vi "test tools list schema details.vi"(8 "error in (no error)":errorcluster) -> (0 "error out":errorcluster, 3 "body":string)   [LabVIEW 2020, in "MCP Server tests.lvlib"]
doc: "tools/list must describe every input completely enough for strict clients such as ChatGPT/Codex. fake_tool_schema_shapes and fake_tool_array_shapes are found by their MCP names, and each kind of input gets its own assertion: a timestamp is a string with format date-time, also as array element; a cluster is an object with properties named by the element labels, nested to any depth and inside arrays; an array of variants (no JSON type) has items {}; a 2D array is an array of arrays; an enum is a string whose enum lists the item names. The request is sent with the LabVIEW HTTP Client directly."
uses:
  MCP Server tests.lvlib
  facb51cd-7822-4ca8-a256-520732c48ef2.vi
  7ce273db-93f1-4574-9673-25cb3b7d48c6.vi
  <vilib>/JDP Science/JSONtext/Next JSON Value.vi
  <vilib>/JDP Science/JSONtext/String Subset.vi
  <vilib>/JDP Science/JSONtext/Parsing/Advance past next JSON Value (inlined COPY).vi
  <vilib>/JDP Science/JSONtext/Parsing/Advance past whitespace.vi
  <vilib>/JDP Science/JSONtext/Parsing/Advance past String.vi
  <vilib>/JDP Science/JSONtext/Parsing/Advance past Number.vi
  <vilib>/JDP Science/JSONtext/Parsing/Advance past Line Ending.vi
  <vilib>/JDP Science/JSONtext/Parsing/Parse Full Path or Item Name.vi
  <vilib>/JDP Science/JSONtext/Parsing/Advance past Array.vi
  <vilib>/JDP Science/JSONtext/Parsing/Advance past Object.vi
  <vilib>/JDP Science/JSONtext/support/Error Cluster From Code.vi
  <vilib>/JDP Science/JSONtext/Offset/Find Item Locations by Path.vi
  <vilib>/JDP Science/JSONtext/JSON text to Variant.vi
  <vilib>/JDP Science/JSONtext/LVClass Serializer/JSONtext LVClass Serializer.lvclass
  <vilib>/addons/_JKI Toolkits/Caraya/classes/Test/Test.lvclass
  <vilib>/JDP Science/JSONtext/JSONtext.lvlib
  <vilib>/addons/_JKI Toolkits/Caraya/classes/Assert/Assert.lvclass
panel:
  out "lookup error":errorcluster
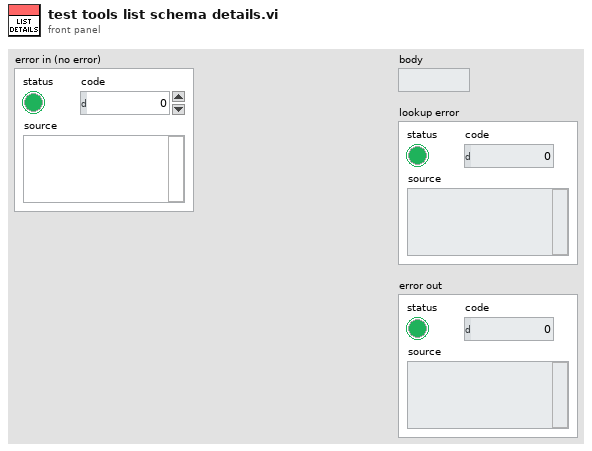
[diagram p1: front panel]
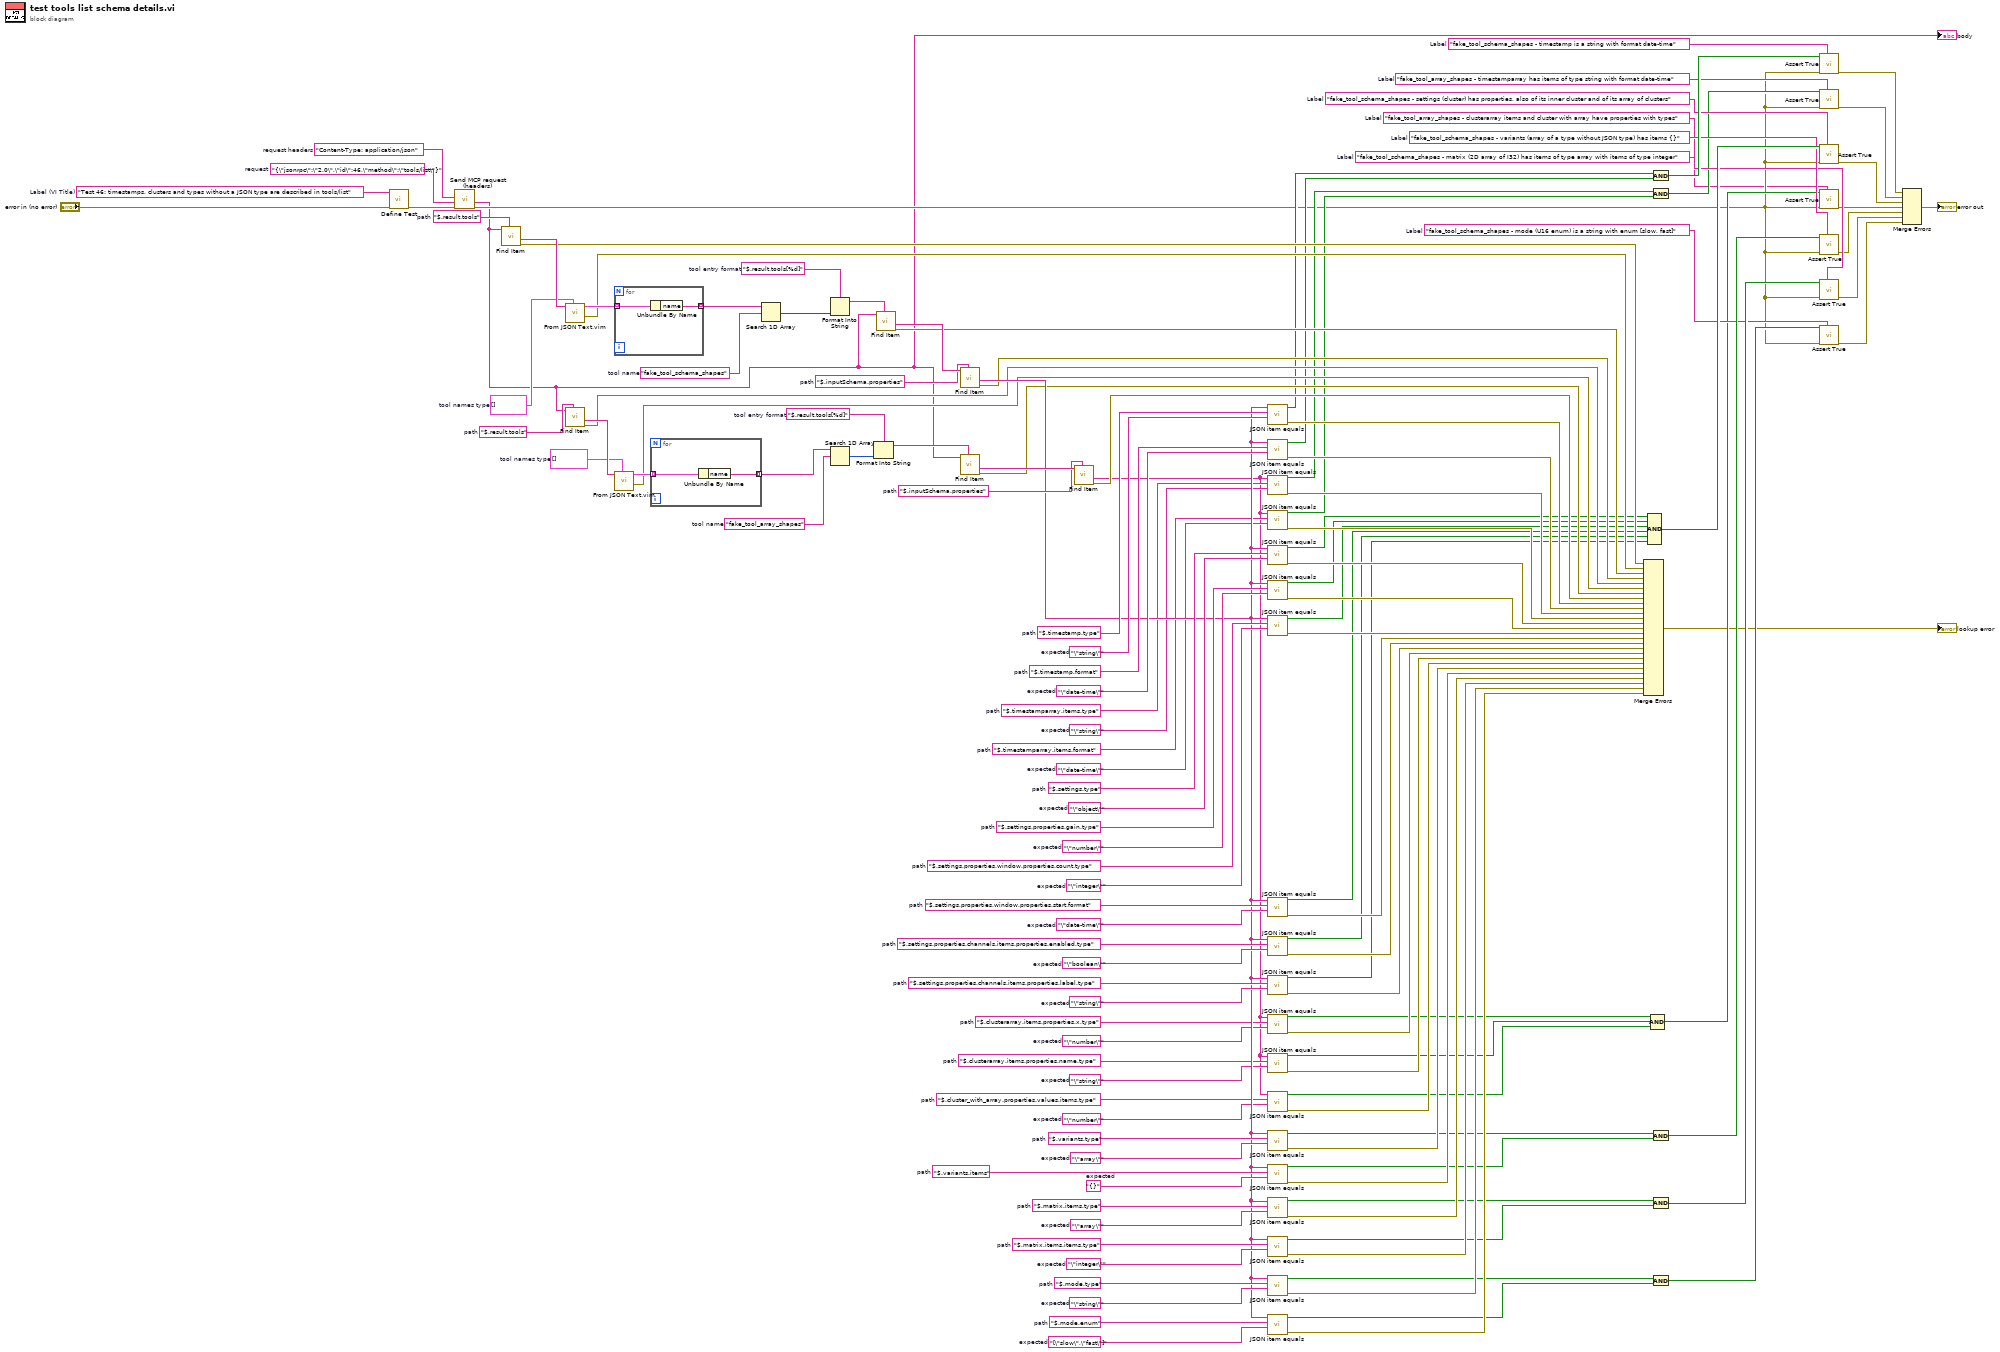
[diagram p0: block diagram]
diagram:
  w136 = "Content-Type: application/json"  # request headers
  w16 = "fake_tool_schema_shapes - mode (U16 enum) is a string with enum [slow, fast]"  # Label
  w18 = "fake_tool_schema_shapes - matrix (2D array of I32) has items of type array with items of type integer"  # Label
  w20 = "fake_tool_schema_shapes - variants (array of a type without JSON type) has items {}"  # Label
  w11 = "fake_tool_array_shapes - clusterarray items and cluster with array have properties with types"  # Label
  w22 = "fake_tool_schema_shapes - settings (cluster) has properties, also of its inner cluster and of its array of clusters"  # Label
  w14 = "fake_tool_array_shapes - timestamparray has items of type string with format date-time"  # Label
  w24 = "fake_tool_schema_shapes - timestamp is a string with format date-time"  # Label
  w83 = "[\"slow\",\"fast\"]"  # expected
  w84 = "$.mode.enum"  # path
  w86 = "\"string\""  # expected
  w87 = "$.mode.type"  # path
  w88 = "\"integer\""  # expected
  w89 = "$.matrix.items.items.type"  # path
  w90 = "\"array\""  # expected
  w91 = "$.matrix.items.type"  # path
  w92 = "{}"  # expected
  w93 = "$.variants.items"  # path
  w94 = "\"array\""  # expected
  w95 = "$.variants.type"  # path
  w46 = "\"number\""  # expected
  w47 = "$.cluster_with_array.properties.values.items.type"  # path
  w75 = "\"string\""  # expected
  w76 = "$.clusterarray.items.properties.name.type"  # path
  w77 = "\"number\""  # expected
  w78 = "$.clusterarray.items.properties.x.type"  # path
  w96 = "\"string\""  # expected
  w97 = "$.settings.properties.channels.items.properties.label.type"  # path
  w98 = "\"boolean\""  # expected
  w99 = "$.settings.properties.channels.items.properties.enabled.type"  # path
  w100 = "\"date-time\""  # expected
  w101 = "$.settings.properties.window.properties.start.format"  # path
  w102 = "\"integer\""  # expected
  w103 = "$.settings.properties.window.properties.count.type"  # path
  w104 = "\"number\""  # expected
  w105 = "$.settings.properties.gain.type"  # path
  w106 = "\"object\""  # expected
  w107 = "$.settings.type"  # path
  w79 = "\"date-time\""  # expected
  w80 = "$.timestamparray.items.format"  # path
  w81 = "\"string\""  # expected
  w82 = "$.timestamparray.items.type"  # path
  w108 = "\"date-time\""  # expected
  w109 = "$.timestamp.format"  # path
  w110 = "\"string\""  # expected
  w111 = "$.timestamp.type"  # path
  w112 = "$.inputSchema.properties"  # path
  w118 = "$.result.tools[%d]"  # tool entry format
  w122 = "fake_tool_array_shapes"  # tool name
  w128 = cluster{"name":string}[] []  # tool names type
  w132 = "$.result.tools"  # path
  w114 = "$.inputSchema.properties"  # path
  w120 = "$.result.tools[%d]"  # tool entry format
  w124 = "fake_tool_schema_shapes"  # tool name
  w130 = cluster{"name":string}[] []  # tool names type
  w133 = "$.result.tools"  # path
  w135 = "{\"jsonrpc\":\"2.0\",\"id\":46,\"method\":\"tools/list\"}"  # request
  w138 = "Test 46: timestamps, clusters and types without a JSON type are described in tools/list"  # Label (VI Title)
  n1 = call <vilib>:"Define Test.vi"("error in (no error)"="error in (no error)", "Label (VI Title)"=w138) -> ("error out"=w134:errorcluster)  [unwired: 8 in, 1 out]
  n2 = call "Send MCP request (headers).vi"("error in (no error)"=w134, "request"=w135, "request headers"=w136) -> ("error out"=w12:errorcluster, "response"=w3:string)  [unwired: 5 in, 2 out]
  "body" <- w3
  n3 = call <vilib>:"Find Item.vi"("$Path or Item Name"=w133, "JSON"=w3) -> ("error out"=w74:errorcluster, "<JSON>"=w131:string)  [unwired: 6 in, 2 out]
  n4 = call "From JSON Text.vim"("Data Type and Default Value"=w130, "JSON"=w131) -> ("error out"=w73:errorcluster, "Data out"=w127:cluster{"name":string}[])  [unwired: 8 in]
  n5 = call <vilib>:"Find Item.vi"("$Path or Item Name"=w132, "JSON"=w3) -> ("error out"=w70:errorcluster, "<JSON>"=w129:string)  [unwired: 6 in, 2 out]
  n6 = for {
    tunnel: w127 -> [w140] mode=indexing
    tunnel: [w139] -> w125 mode=indexing
    n7 = Unbundle By Name(w140) -> ("name"=w139:string)
  }
  n8 = call "From JSON Text.vim"("Data Type and Default Value"=w128, "JSON"=w129) -> ("error out"=w69:errorcluster, "Data out"=w126:cluster{"name":string}[])  [unwired: 8 in]
  n9 = for {
    tunnel: w126 -> [w142] mode=indexing
    tunnel: [w141] -> w123 mode=indexing
    n10 = Unbundle By Name(w142) -> ("name"=w141:string)
  }
  n11 = Search 1D Array(1D array=w125, element=w124) -> (index of element=w121:i32)  [unwired: 1 in]
  n12 = Format Into String(format string=w120, w121) -> (resulting string=w117:string)  [unwired: 2 in, 1 out]
  n13 = Search 1D Array(1D array=w123, element=w122) -> (index of element=w119:i32)  [unwired: 1 in]
  n14 = Format Into String(format string=w118, w119) -> (resulting string=w116:string)  [unwired: 2 in, 1 out]
  n15 = call <vilib>:"Find Item.vi"("$Path or Item Name"=w117, "JSON"=w3) -> ("error out"=w72:errorcluster, "<JSON>"=w115:string)  [unwired: 6 in, 2 out]
  n16 = call <vilib>:"Find Item.vi"("$Path or Item Name"=w114, "JSON"=w115) -> ("error out"=w71:errorcluster, "<JSON>"=w85:string)  [unwired: 6 in, 2 out]
  n17 = call <vilib>:"Find Item.vi"("$Path or Item Name"=w116, "JSON"=w3) -> ("error out"=w68:errorcluster, "<JSON>"=w113:string)  [unwired: 6 in, 2 out]
  n18 = call <vilib>:"Find Item.vi"("$Path or Item Name"=w112, "JSON"=w113) -> ("error out"=w67:errorcluster, "<JSON>"=w48:string)  [unwired: 6 in, 2 out]
  n19 = call "JSON item equals.vi"("expected"=w110, "path"=w111, "JSON"=w85) -> ("error out"=w66:errorcluster, "equal?"=w44:bool)  [unwired: 6 in, 1 out]
  n20 = call "JSON item equals.vi"("expected"=w108, "path"=w109, "JSON"=w85) -> ("error out"=w65:errorcluster, "equal?"=w43:bool)  [unwired: 6 in, 1 out]
  n21 = call "JSON item equals.vi"("expected"=w81, "path"=w82, "JSON"=w48) -> ("error out"=w64:errorcluster, "equal?"=w30:bool)  [unwired: 6 in, 1 out]
  n22 = call "JSON item equals.vi"("expected"=w79, "path"=w80, "JSON"=w48) -> ("error out"=w63:errorcluster, "equal?"=w29:bool)  [unwired: 6 in, 1 out]
  n23 = call "JSON item equals.vi"("expected"=w106, "path"=w107, "JSON"=w85) -> ("error out"=w62:errorcluster, "equal?"=w42:bool)  [unwired: 6 in, 1 out]
  n24 = call "JSON item equals.vi"("expected"=w104, "path"=w105, "JSON"=w85) -> ("error out"=w61:errorcluster, "equal?"=w41:bool)  [unwired: 6 in, 1 out]
  n25 = call "JSON item equals.vi"("expected"=w102, "path"=w103, "JSON"=w85) -> ("error out"=w60:errorcluster, "equal?"=w40:bool)  [unwired: 6 in, 1 out]
  n26 = call "JSON item equals.vi"("expected"=w100, "path"=w101, "JSON"=w85) -> ("error out"=w59:errorcluster, "equal?"=w39:bool)  [unwired: 6 in, 1 out]
  n27 = call "JSON item equals.vi"("expected"=w98, "path"=w99, "JSON"=w85) -> ("error out"=w58:errorcluster, "equal?"=w38:bool)  [unwired: 6 in, 1 out]
  n28 = call "JSON item equals.vi"("expected"=w96, "path"=w97, "JSON"=w85) -> ("error out"=w57:errorcluster, "equal?"=w37:bool)  [unwired: 6 in, 1 out]
  n29 = call "JSON item equals.vi"("expected"=w77, "path"=w78, "JSON"=w48) -> ("error out"=w56:errorcluster, "equal?"=w28:bool)  [unwired: 6 in, 1 out]
  n30 = call "JSON item equals.vi"("expected"=w75, "path"=w76, "JSON"=w48) -> ("error out"=w55:errorcluster, "equal?"=w27:bool)  [unwired: 6 in, 1 out]
  n31 = call "JSON item equals.vi"("expected"=w46, "path"=w47, "JSON"=w48) -> ("error out"=w45:errorcluster, "equal?"=w26:bool)  [unwired: 6 in, 1 out]
  n32 = call "JSON item equals.vi"("expected"=w94, "path"=w95, "JSON"=w85) -> ("error out"=w54:errorcluster, "equal?"=w36:bool)  [unwired: 6 in, 1 out]
  n33 = call "JSON item equals.vi"("expected"=w92, "path"=w93, "JSON"=w85) -> ("error out"=w53:errorcluster, "equal?"=w35:bool)  [unwired: 6 in, 1 out]
  n34 = call "JSON item equals.vi"("expected"=w90, "path"=w91, "JSON"=w85) -> ("error out"=w52:errorcluster, "equal?"=w34:bool)  [unwired: 6 in, 1 out]
  n35 = call "JSON item equals.vi"("expected"=w88, "path"=w89, "JSON"=w85) -> ("error out"=w51:errorcluster, "equal?"=w33:bool)  [unwired: 6 in, 1 out]
  n36 = call "JSON item equals.vi"("expected"=w86, "path"=w87, "JSON"=w85) -> ("error out"=w50:errorcluster, "equal?"=w32:bool)  [unwired: 6 in, 1 out]
  n37 = call "JSON item equals.vi"("expected"=w83, "path"=w84, "JSON"=w85) -> ("error out"=w49:errorcluster, "equal?"=w31:bool)  [unwired: 6 in, 1 out]
  n38 = Merge Errors(w74, w73, w72, w71, w70, w69, w68, w67, w66, w65, w64, w63, w62, w61, w60, w59, w58, w57, w56, w55, w45, w54, w53, w52, w51, w50, w49) -> (→"lookup error":errorcluster)
  n39 = Compound Arithmetic op=AND(w42, w41, w40, w39, w38, w37) -> (w23:bool)
  n40 = Compound Arithmetic op=AND(w28, w27, w26) -> (w13:bool)
  n41 = Compound Arithmetic op=AND(w44, w43) -> (w25:bool)
  n42 = Compound Arithmetic op=AND(w30, w29) -> (w15:bool)
  n43 = Compound Arithmetic op=AND(w36, w35) -> (w21:bool)
  n44 = Compound Arithmetic op=AND(w34, w33) -> (w19:bool)
  n45 = Compound Arithmetic op=AND(w32, w31) -> (w17:bool)
  n46 = call <vilib>:"Assert True.vi"("Label"=w24, "error in (no error)"=w12, "True?"=w25) -> ("error out"=w10:errorcluster)  [unwired: 7 in, 1 out]
  n47 = call <vilib>:"Assert True.vi"("Label"=w14, "error in (no error)"=w12, "True?"=w15) -> ("error out"=w9:errorcluster)  [unwired: 7 in, 1 out]
  n48 = call <vilib>:"Assert True.vi"("Label"=w22, "error in (no error)"=w12, "True?"=w23) -> ("error out"=w8:errorcluster)  [unwired: 7 in, 1 out]
  n49 = call <vilib>:"Assert True.vi"("Label"=w11, "error in (no error)"=w12, "True?"=w13) -> ("error out"=w7:errorcluster)  [unwired: 7 in, 1 out]
  n50 = call <vilib>:"Assert True.vi"("Label"=w20, "error in (no error)"=w12, "True?"=w21) -> ("error out"=w6:errorcluster)  [unwired: 7 in, 1 out]
  n51 = call <vilib>:"Assert True.vi"("Label"=w18, "error in (no error)"=w12, "True?"=w19) -> ("error out"=w5:errorcluster)  [unwired: 7 in, 1 out]
  n52 = call <vilib>:"Assert True.vi"("Label"=w16, "error in (no error)"=w12, "True?"=w17) -> ("error out"=w4:errorcluster)  [unwired: 7 in, 1 out]
  n53 = Merge Errors(w10, w9, w8, w7, w6, w5, w4) -> (→"error out":errorcluster)
